vi "Mass Compile CalcExpress VIs.vi"() -> ()   [LabVIEW 2021]
doc: "This utility assists in compiling all CalcExpress VIs in bulk, including examples, utilities, and templates.\n\n::: CalcExpress Toolkit :::\nCopyright (c) 2000-2026 Konstantin Shifershteyn. All rights reserved."
uses:
  <vilib>/event_ctls.llb/eventvkey.ctl
  vi.lib/addons/CalcExpress/cemisc.llb/[ce] CE component paths - Kind of Path Enum.ctl
panel:
  in  "Open Logfile":bool
  in  "<Templates>":bool=TRUE caption="CalcExpress VIs in <Templates>"
  in  "Cache VIs":u32=20
  in  "Compile":bool
  in  "Exit":bool
  in  "Log mode":T1(ring)
  in  "Log file":path
  in  "<Examples>":bool=TRUE caption="CalcExpress VIs in <Examples>"
  in  "<Project>":bool=TRUE caption="CalcExpress VIs in <Project>"
  in  "<vi.lib>":bool=TRUE caption="CalcExpress VIs in <vi.lib>"
  # "Compile parameters"
  # "Compiling log file"
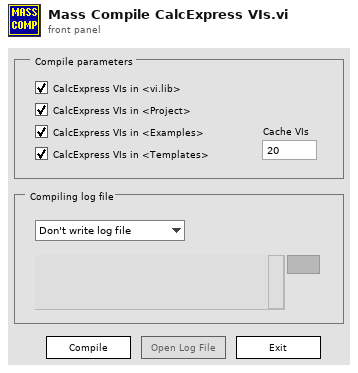
[diagram p1: front panel]
types:
  T1 = enum16{"Don't write log file", "Write new log file", "Append to log file"}
  T2 = typedef "eventvkey.ctl" = enum16{"ASCII", "Enter", "Return", "Shift", "Ctrl", "Alt", "Cmd", "Opt", "Caps", "NumLock", "Clear", "Break", "Up", "Down", "Left", "Right", "Insert", "Delete", "Home", "End", "PageUp", "PageDown", "Escape", "Help", "Pause", "ScrollLock", "F1", "F2", "F3", "F4", "F5", "F6", "F7", "F8", "F9", "F10", "F11", "F12", "F13", "F14", "F15", "F16", "F17", "F18", "F19", "F20", "F21", "F22", "F23", "F24", "Play", "VolumeUp", "VolumeDown", "Mute", "Two Byte Char"}
  T3 = cluster{"Shift":bool, "Ctrl":bool, "Alt":bool, "Cmd":bool, "Opt":bool}
  T4 = typedef "[ce] CE component paths - Kind of Path Enum.ctl" = enum16{"VIs", "FuncVIs", "Help", "Examples", "Project", "Templates"}
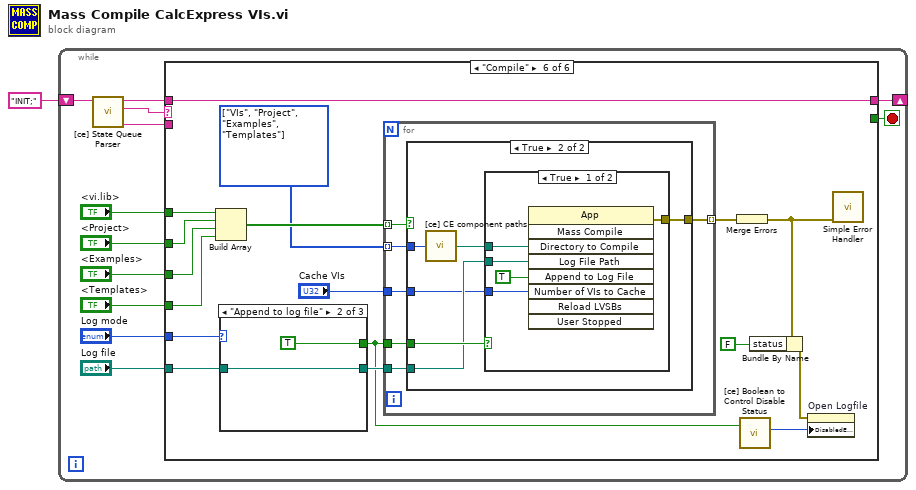
[diagram p0: block diagram]
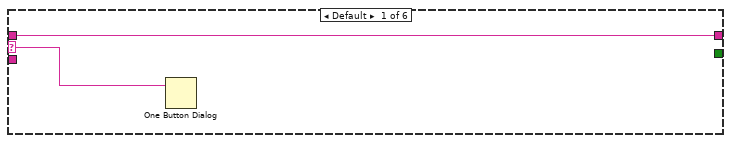
[diagram p2: hidden frame]
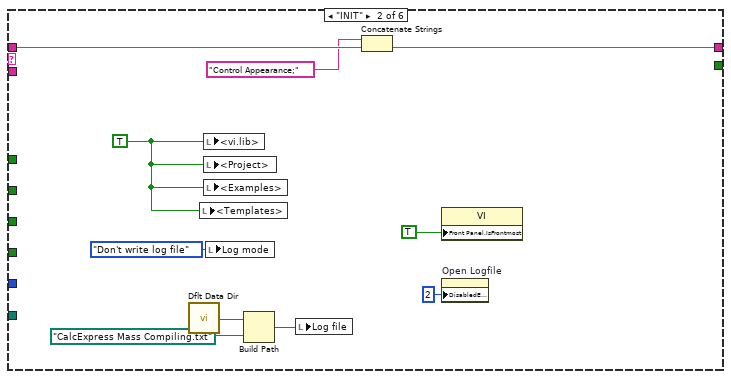
[diagram p3: hidden frame]
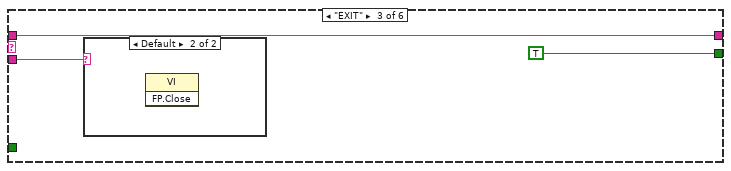
[diagram p4: hidden frame]
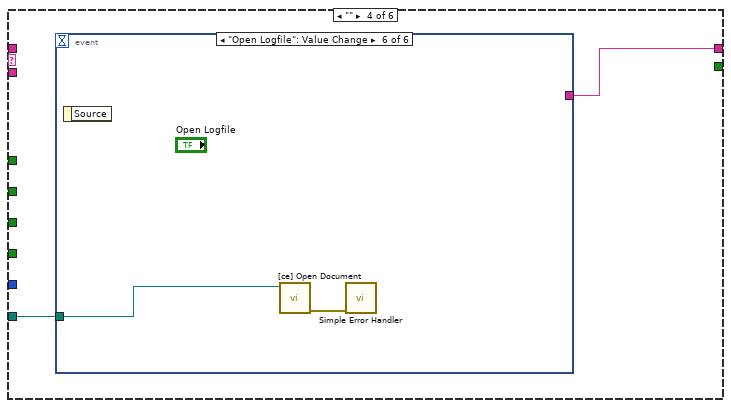
[diagram p6: hidden frame]
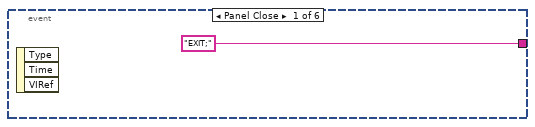
[diagram p7: hidden frame]
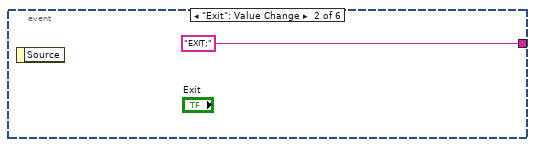
[diagram p8: hidden frame]
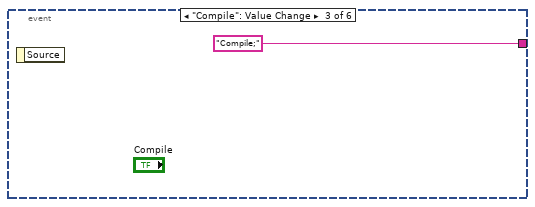
[diagram p9: hidden frame]
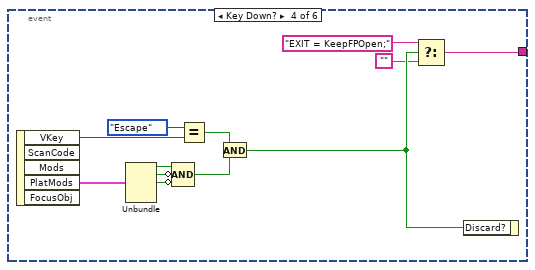
[diagram p10: hidden frame]
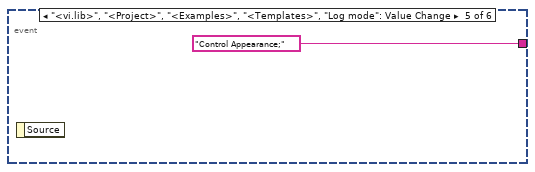
[diagram p11: hidden frame]
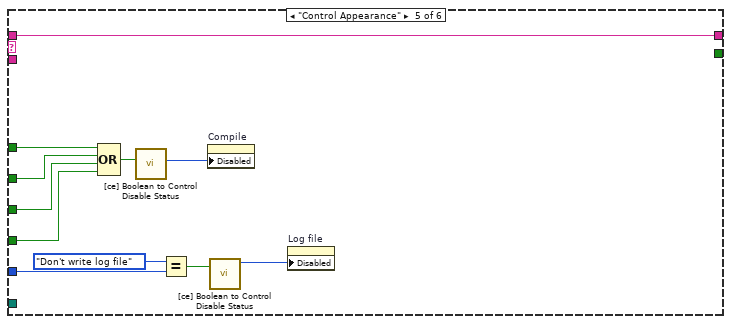
[diagram p12: hidden frame]
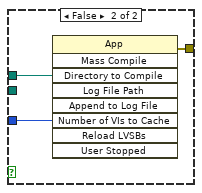
[diagram p14: hidden frame]
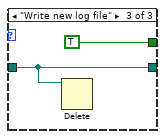
[diagram p16: hidden frame]
diagram:
  n1 = while {
    shift-right: [w13] -> _
    shift-left: "INIT;" -> [w6]
    stop <- w12 stop-if-true
    n2 = call "[ce] State Queue Parser.vi"("input queue"=w6) -> ("state parameters"=w3:string, "state"=w4:string, "remained queue"=w5:string)  [unwired: 6 in]
    n3 = case shown="\"Compile\"" w4 {
      selector: w4 -> [w14 _ _ _ _ _]
      tunnel: w5 -> [w15 w22 w28 _ w59 w76]
      tunnel: [w15 w21 w28 w30 w59 w76] -> w13
      tunnel: [_ _ TRUE _ _ _] -> w12
      tunnel: "<vi.lib>" -> [_ _ _ _ w58 w73]
      tunnel: "<Project>" -> [_ _ _ _ w57 w72]
      tunnel: "<Examples>" -> [_ _ _ _ w56 w71]
      tunnel: "Log mode" -> [_ _ _ _ w55 w75]
      tunnel: "Log file" -> [_ _ _ w29 _ w74]
      tunnel: w3 -> [_ _ w26 _ _ _]
      tunnel: "<Templates>" -> [_ _ _ _ w49 w66]
      frame Default {
        n4 = One Button Dialog(message=w14) -> ()  [unwired: 1 in, 1 out]
      }
      frame "INIT" {
        w18 = TRUE ("CalcExpress VIs in <vi.lib>")
        n5 = call <vilib>:"Dflt Data Dir.vi"() -> ("App:Default Data Directory"=w16:path)
        n6 = local write "<Templates>"(w18) -> ()
        n7 = local write "<vi.lib>"(w18) -> ()
        n8 = local write "<Project>"(w18) -> ()
        n9 = local write "<Examples>"(w18) -> ()
        n10 = local write "Log mode"(T1."Don't write log file" ("Log mode")) -> ()
        n11 = Build Path(base path=w16, name or relative path=path "CalcExpress Mass Compiling.txt") -> (appended path=w25:path)
        n12 = local write "Log file"(w25) -> ()
        n13 = Concatenate Strings("Control Appearance;", w22) -> (w21:string)
        n14 = property class="VI"("Front Panel.IsFrontmost"=TRUE) -> ()  [unwired: 2 in, 2 out]
        n15 = property on="Open Logfile" class="Bool"("DisabledEnum"=u8 2 ("Control Disable if False")) -> ()  [unwired: 2 in, 2 out]
      }
      frame "EXIT" {
        n16 = case shown="Default" w26 {
          frame "KeepFPOpen" {
          }
          frame Default {
            n17 = invoke class="VI" method="FP.Close"() -> ()  [unwired: 3 in, 3 out]
          }
        }
      }
      frame "" {
        n18 = event shown="[5] \"Open Logfile\": Value Change" {
          selector: _ -> [_ _ _ _ _ _]
          dyn-events: _ -> [_ _ _ _ _ _]
          timeout: _ -> [_ _ _ _ _ _]
          tunnel: ["EXIT;" "EXIT;" "Compile;" w36 "Control Appearance;" _] -> w30
          tunnel: w29 -> [_ _ _ _ _ w48]
          event Panel Close {
            n19 = event-data() -> ()  [unwired: 1 in, 3 out]
          }
          event "Exit": Value Change {
            n20 = event-data() -> ()  [unwired: 1 in, 1 out]
          }
          event "Compile": Value Change {
            n21 = event-data() -> ()  [unwired: 1 in, 1 out]
          }
          event Key Down? {
            n22 = event-data() -> ("VKey"=w44:T2, "PlatMods"=w45:T3)  [unwired: 1 in, 3 out]
            n23 = Unbundle(w45) -> ("Shift"=w42:bool, "Ctrl"=w41:bool, "Alt"=w40:bool)  [unwired: 2 out]
            n24 = Compound Arithmetic op=AND(w42, invert w41, invert w40) -> (w39:bool)
            n25 = Equal?(x=eventvkey."Escape", y=w44) -> (x = y?=w38:bool)
            n26 = And(x=w38, y=w39) -> (x .and. y?=w37:bool)
            n27 = Select(t="EXIT = KeepFPOpen;", s=w37, f="") -> (s? t:f=w36:string)
            n28 = event-data("Discard?"=w37) -> ()  [unwired: 1 in, 1 out]
          }
          event "<vi.lib>", "<Project>", "<Examples>", "<Templates>", "Log mode": Value Change {
            n29 = event-data() -> ()  [unwired: 1 in, 1 out]
          }
          event "Open Logfile": Value Change {
            n30 = event-data() -> ()  [unwired: 1 in, 1 out]
            n31 = call "[ce] Open Document.vi"("file path"=w48) -> ("error out"=w47:errorcluster)  [unwired: 10 in]
            n32 = call <vilib>:"Simple Error Handler.vi"("error in (no error)"=w47) -> ()  [unwired: 4 in, 5 out]
          }
        }
      }
      frame "Control Appearance" {
        n33 = Compound Arithmetic op=OR(w58, w57, w56, w49) -> (w53:bool)
        n34 = call "[ce] Boolean to Control Disable Status.vi"("Status in"=w53) -> ("Control Disable if False"=w52:u8)  [unwired: 3 in, 1 out]
        n35 = Equal?(x=T1."Don't write log file", y=w55) -> (x = y?=w51:bool)
        n36 = property on="Compile" class="Bool"("Disabled"=w52) -> ()  [unwired: 2 in, 2 out]
        n37 = call "[ce] Boolean to Control Disable Status.vi"("Status in"=w51) -> ("Control Disable if True"=w50:u8)  [unwired: 3 in, 1 out]
        n38 = property on="Log file" class="Path"("Disabled"=w50) -> ()  [unwired: 2 in, 2 out]
      }
      frame "Compile" {
        w65 = T4[] [enum."VIs", enum."Project", enum."Examples", enum."Templates"] items=["VIs", "FuncVIs", "Help", "Examples", "Project", "Templates"]
        n39 = Build Array(w73, w72, w71, w66) -> (w70:bool[])
        n40 = case shown="\"Append to log file\"" w75 {
          tunnel: w74 -> [_ w98 w100]
          tunnel: [_ w98 w100] -> w69
          tunnel: [_ TRUE TRUE] -> w64
          frame "Don't write log file" {
          }
          frame "Append to log file" {
          }
          frame "Write new log file" {
            n41 = Delete(path (use dialog)=w100) -> ()  [unwired: 4 in, 3 out]
          }
        }
        n42 = for {
          tunnel: w70 -> [w82] mode=indexing
          tunnel: w64 -> [w81]
          tunnel: w69 -> [w80]
          tunnel: [w79] -> w68 mode=indexing
          tunnel: "Cache VIs" -> [w78]
          tunnel: w65 -> [w77] mode=indexing
          n43 = case shown="True" w82 {
            tunnel: w81 -> [_ w87]
            tunnel: w80 -> [_ w86]
            tunnel: [_ w85] -> w79
            tunnel: w78 -> [_ w84]
            tunnel: w77 -> [_ w83]
            frame False {
            }
            frame True {
              n44 = call "[ce] CE component paths.vi"("kind of path"=w83) -> ("path out"=w88:path)  [unwired: 1 in]
              n45 = case shown="True" w87 {
                tunnel: w88 -> [w93 w96]
                tunnel: w86 -> [w92 _]
                tunnel: [w90 w95] -> w85
                tunnel: w84 -> [w89 w94]
                frame True {
                  n46 = invoke class="App" method="Mass Compile"("Directory to Compile"=w93, "Log File Path"=w92, "Append to Log File"=TRUE, "Number of VIs to Cache"=w89) -> (error out=w90:errorcluster)  [unwired: 5 in, 8 out]
                }
                frame False {
                  n47 = invoke class="App" method="Mass Compile"("Directory to Compile"=w96, "Number of VIs to Cache"=w94) -> (error out=w95:errorcluster)  [unwired: 7 in, 8 out]
                }
              }
            }
          }
        }
        n48 = Merge Errors(w68) -> (w62:errorcluster)
        n49 = call "[ce] Boolean to Control Disable Status.vi"("Status in"=w64) -> ("Control Disable if False"=w63:u8)  [unwired: 3 in, 1 out]
        n50 = Bundle By Name(cluster=w62, "status"=FALSE) -> (w61:errorcluster)
        n51 = property on="Open Logfile" class="Bool"(error in=w61, "DisabledEnum"=w63) -> ()  [unwired: 1 in, 2 out]
        n52 = call <vilib>:"Simple Error Handler.vi"("error in (no error)"=w62) -> ()  [unwired: 4 in, 5 out]
      }
    }
  }
